vi "CompVisionUtil_EstimateFieldToRobot_Alt.vi"(9 "CameraToRobot":T1={"TRANSLATION3D"={"X"=0.0, "Y"=0.0, "Z"=0.0}, "ROTATION3D"={"Q_quaternion"={"R"=1.0, "V"=[0.0, 0.0, 0.0]}}, "XF"=FALSE} {"TRANSLATION3D"."Z" format="%14.3f"; "TRANSLATION3D"."Y" format="%14.3f"; "TRANSLATION3D"."X" format="%14.3f"}, 10 "FieldToTarget":T5={"Translation3d"={"X"=0.0, "Y"=0.0, "Z"=0.0}, "Rotation3d"={"Q_quaternion"={"R"=1.0, "V"=[0.0, 0.0, 0.0]}}} {"Translation3d"."Z" format="%14.3f"; "Translation3d"."Y" format="%14.3f"; "Translation3d"."X" format="%14.3f"}, 11 "CameraToTarget":T1={"TRANSLATION3D"={"X"=0.0, "Y"=0.0, "Z"=0.0}, "ROTATION3D"={"Q_quaternion"={"R"=1.0, "V"=[0.0, 0.0, 0.0]}}, "XF"=FALSE} {"TRANSLATION3D"."Z" format="%14.3f"; "TRANSLATION3D"."Y" format="%14.3f"; "TRANSLATION3D"."X" format="%14.3f"}) -> (3 "EstimatedFieldToRobot":T5={"Translation3d"={"X"=0.0, "Y"=0.0, "Z"=0.0}, "Rotation3d"={"Q_quaternion"={"R"=1.0, "V"=[0.0, 0.0, 0.0]}}} {"Translation3d"."Z" format="%14.3f"; "Translation3d"."Y" format="%14.3f"; "Translation3d"."X" format="%14.3f"})   [LabVIEW 2019, in "Trajectory_Library.lvlib"]
doc: "Estimates the pose of the robot in the field coordinate system, given the position of the target relative to the camera, the target relative to the field, and the robot relative to the camera.\n\nInputs:\n -- CameraToTarget -- Transform3d containing the position of the target relative to the camera.\n -- FieldToTarget -- Pose3d containing the position of the target in the field.\n -- CameraToRobot -- Transform3d containing the position of the robot relative to the camera. If the camera was mounted 3 inches behind the \"origin\" (usually physical center) of the robot, this would be Transform2d(3 inches, 0 inches, 0 inches, 0 degrees).\n\nOutput:\n -- EstimatedFieldToRobot -- A Pose3d containing the position of the robot in the field."
uses:
  Trajectory_Library.lvlib
  TypeDef/TRANSLATION3D.ctl
  TypeDef/QUATERNION.ctl
  TypeDef/ROTATION3D.ctl
  TypeDef/TRANSFORM3D.ctl
  TypeDef/POSE3D.ctl
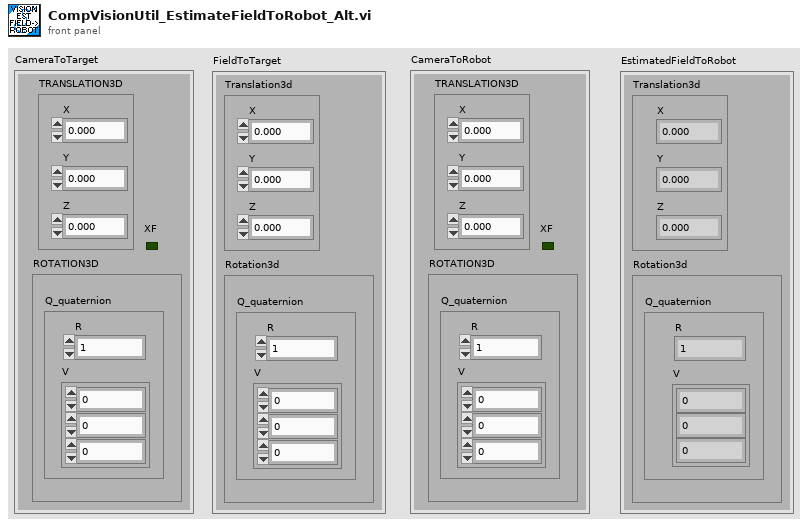
[diagram p1: front panel]
types:
  T1 = typedef "Trajectory_Library.lvlib/TRANSFORM3D.ctl" = cluster{"TRANSLATION3D":T2, "ROTATION3D":T3, "XF":bool}
  T2 = typedef "Trajectory_Library.lvlib/TRANSLATION3D.ctl" = cluster{"X":dbl, "Y":dbl, "Z":dbl}
  T3 = typedef "Trajectory_Library.lvlib/ROTATION3D.ctl" = cluster{"Q_quaternion":T4}
  T4 = typedef "Trajectory_Library.lvlib/QUATERNION.ctl" = cluster{"R":dbl, "V":dbl[]}
  T5 = typedef "Trajectory_Library.lvlib/POSE3D.ctl" = cluster{"Translation3d":T2, "Rotation3d":T3}
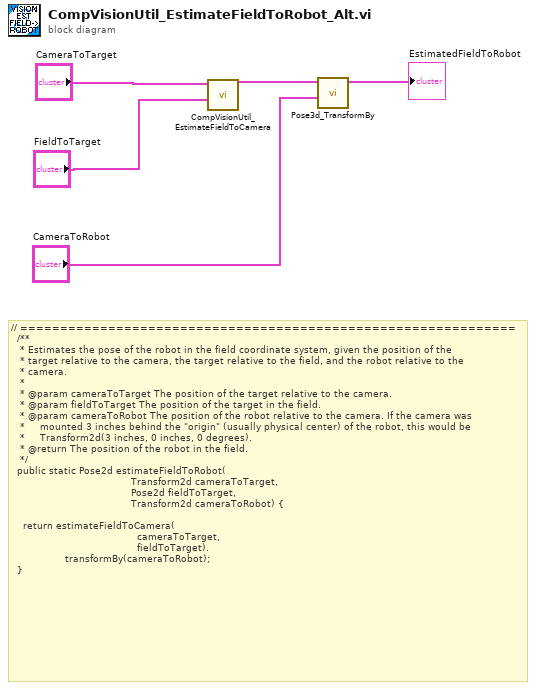
[diagram p0: block diagram]
diagram:
  # "// ==============================================================\n  /**\n   * Estimates the pose of the robot in the field coordinate system, given the position of the\n   * target relative to the camera, the target relative to the field, and the robot relative to the\n   * camera.\n   *\n   * @param cameraToTarget The position of the target relative to the camera.\n   * @param fieldToTarget The position of the target in the field.\n   * @param cameraToRobot The position of the robot relative to the camera. If the camera was\n   *     mounted 3 inches behind the \"origin\" (usually physical center) of the robot, this would be\n   *     Transform2d(3 inches, 0 inches, 0 degrees).\n   * @return The position of the robot in the field.\n   */\n  public static Pose2d estimateFieldToRobot(\n                                        Transform2d cameraToTarget, \n                                        Pose2d fieldToTarget, \n                                        Transform2d cameraToRobot) {\n\n    return estimateFieldToCamera(\n                                          cameraToTarget, \n                                          fieldToTarget).\n                  transformBy(cameraToRobot);\n  }"
  n1 = call "CompVisionUtil_EstimateFieldToCamera.vi"("FieldToTarget"="FieldToTarget", "CameraToTarget"="CameraToTarget") -> ("EstimateFieldToCamera"=w3:T5)  [unwired: 9 in]
  n2 = call "Pose3d_TransformBy.vi"("other Transform3d"="CameraToRobot", "in Pose3d"=w3) -> ("out POSE3d"=→"EstimatedFieldToRobot":T5)  [unwired: 9 in]
